vi "CANsub_REST_Open.vi"(8 "error in (no error)":errorcluster, 11 "cert path":path) -> (0 "error out":errorcluster, 3 "client handle":T1)   [LabVIEW 2021, in "CANsub_Common.lvlib"]
uses:
  CANsub_Common.lvlib
  <vilib>/httpClient/LabVIEWHTTPClient.lvlib
  <vilib>/httpClient/ClientHandle.ctl
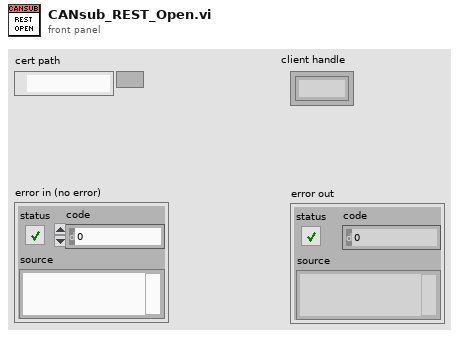
[diagram p1: front panel]
types:
  T1 = typedef "LabVIEWHTTPClient.lvlib/ClientHandle.ctl" = refnum<k1>
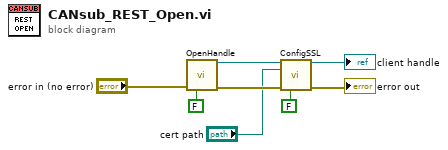
[diagram p0: block diagram]
diagram:
  n1 = call <vilib>:"OpenHandle.vi"("error in (no error)"="error in (no error)", "verify server(true)"=FALSE) -> ("client handle out"=w5:T1, "error out"=w7:errorcluster)  [unwired: 12 in]
  n2 = call <vilib>:"ConfigSSL.vi"("client handle"=w5, "CA certificate file"="cert path", "error in (no error)"=w7, "verify server (true)"=FALSE) -> ("client handle out"=→"client handle":T1, "error out"=→"error out":errorcluster)  [unwired: 10 in]
